vi "Trajektorie.vi"(10 "StateIn":dbl[](array[numeric])=[0.0, 0.0, 0.0, 0.0, 0.0, 0.0, 0.0, 0.0, 0.0, 0.0, 0.0, 0.0], 11 "Parameters":dbl[](array[numeric])=[0.05, 0.0, 20.0, 2.0, 0.5, 1.0, 0.0, 0.0, 0.0, 0.0, 0.0, 0.5, 0.0]) -> (2 "Values":dbl[](array[numeric]), 3 "StateOut":dbl[](array[numeric]))   [LabVIEW 2026]
doc: "AT1B virtual sensor workbench: deterministic model step. Explicit state, no hardware access. See model contract and assumptions."
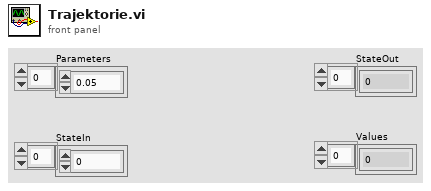
[diagram p1: front panel]
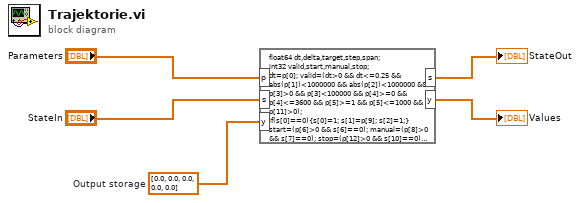
[diagram p0: block diagram]
diagram:
  w3 = dbl[] [0.0, 0.0, 0.0, 0.0, 0.0]  # Output storage
  n1 = formula code="float64 dt,delta,target,step,span;\nint32 valid,start,manual,stop;\ndt=p[0]; valid=(dt>0 && dt<=0.25 && abs(p[1])<1000000 && abs(p[2])<1000000 && p[3]>0 && p[3]<100000 && p[4]>=0 && p[4]<=3600 && p[5]>=1 && p[5]<=1000 && p[11]>0);\nif(s[0]==0){s[0]=1; s[1]=p[9]; s[2]=1;}\nstart=(p[6]>0 && s[6]==0); manual=(p[8]>0 && s[7]==0); stop=(p[12]>0 && s[10]==0);\nif(valid){\n  s[8]=s[8]+dt;\n  if(start){s[1]=p[1]; s[2]=1; if(p[2]<p[1]){s[2]=-1;} s[3]=1; s[4]=0; s[5]=0; s[9]=1;}\n  if(manual && abs(p[9])<1000000){s[1]=p[9]; s[3]=0;}\n  if(stop){s[3]=0;}\n  if(s[3]>0 && p[7]==0){\n    if(s[5]>0){s[5]=s[5]-dt; if(s[5]<0){s[5]=0;}}\n    else {\n      target=p[2]; if(s[9]==0){target=p[1];}\n      delta=target-s[1]; step=p[3]*dt;\n      if(p[10]==1){step=p[11];}\n      if(abs(delta)<=step){\n        s[1]=target; s[5]=p[4];\n        if(p[10]==2){s[3]=0; s[4]=1;}\n        else {if(s[9]>0){s[9]=0; s[2]=-s[2];} else {s[4]=s[4]+1; if(s[4]>=floor(p[5])){s[3]=0;} else {s[9]=1; s[2]=-s[2];}}}\n      } else {if(delta>0){s[1]=s[1]+step;} else {s[1]=s[1]-step;} if(p[10]==1){s[5]=p[4];}}\n    }\n  }\n}\ns[6]=(p[6]>0); s[7]=(p[8]>0); s[10]=(p[12]>0);\ny[0]=s[1]; y[1]=s[3]; y[2]=s[4]; y[3]=s[8]; y[4]=valid;"("p"="Parameters", "s"="StateIn", "y"=w3) -> ("s"=→"StateOut":dbl[], "y"=→"Values":dbl[])
